vi "RT_NetworkStreams.vi"() -> ()   [LabVIEW 2025]
uses:
  <vilib>/dex/Flush And Wait Empty Condition.ctl
panel:
  out "error out 2":errorcluster
  out "error out":errorcluster
  out "Sinus RT":dbl[](graph)
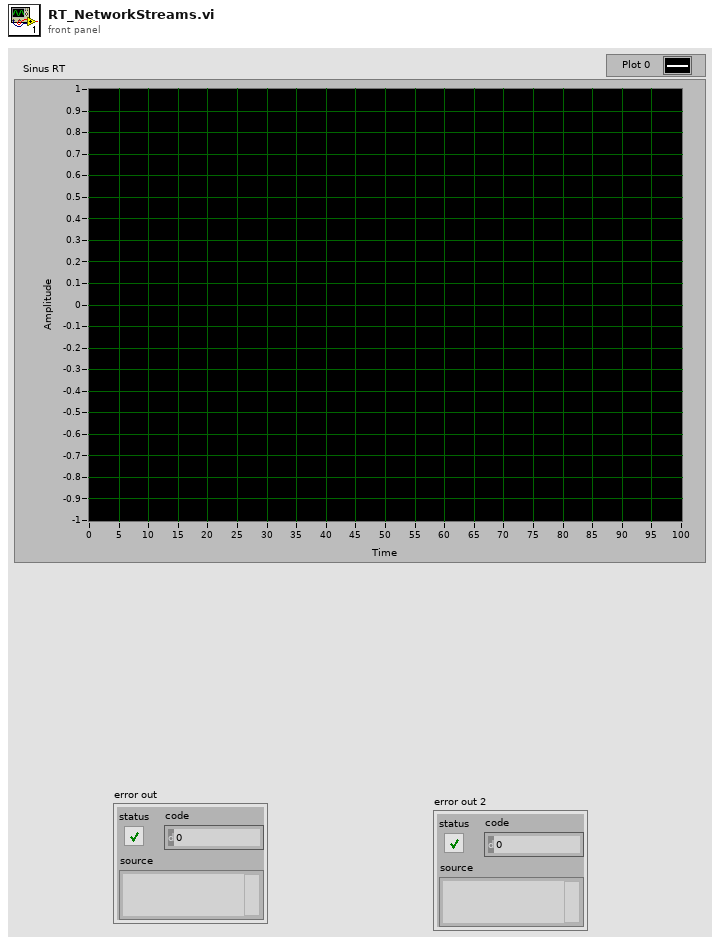
[diagram p1: front panel]
types:
  T1 = typedef "Flush And Wait Empty Condition.ctl" = u8
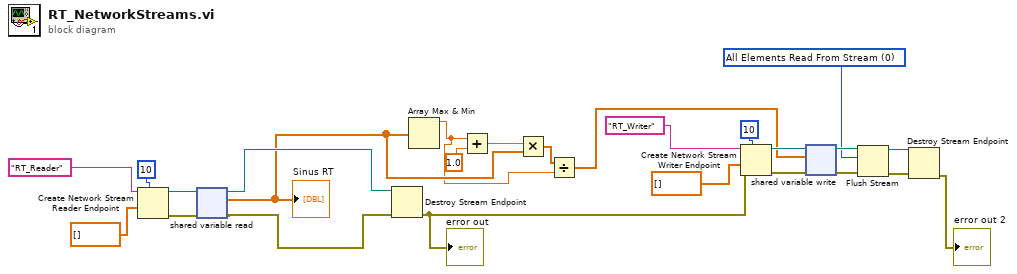
[diagram p0: block diagram]
diagram:
  w7 = T1 0 items=["All Elements Read From Stream", "All Elements Available for Reading"] ("wait condition")
  n1 = Create Network Stream Reader Endpoint(7:10 ("reader buffer size"), 9:dbl[] [], 11:"RT_Reader" ("reader name")) -> (0:w21:errorcluster, 3:w22:refnum<k21>)  [unwired: 4 in]
  n2 = shared-variable-read(w22, w21) -> (w20:refnum<k21>, w19:errorcluster, w4:dbl[])  [unwired: 1 in, 1 out]
  "Sinus RT" <- w4
  n3 = Destroy Stream Endpoint(8:w19, 11:w20) -> (0:w18:errorcluster)
  "error out" <- w18
  n4 = Array Max & Min(array=w4) -> (max value=w2:dbl)  [unwired: 3 out]
  n5 = Add(x=w2, y=1.0) -> (x+y=w5:dbl)
  n6 = Multiply(x=w5, y=w4) -> (x*y=w3:dbl[])
  n7 = Divide(x=w3, y=w2) -> (x/y=w1:dbl[])
  n8 = Create Network Stream Writer Endpoint(7:10 ("writer buffer size"), 8:w18, 9:dbl[] [], 11:"RT_Writer" ("writer name")) -> (0:w13:errorcluster, 3:w14:refnum<k21>)  [unwired: 3 in]
  n9 = shared-variable-write(w14, w13, w1) -> (w11:refnum<k21>, w12:errorcluster)  [unwired: 1 in, 1 out]
  n10 = Flush Stream(8:w12, 10:w7, 11:w11) -> (0:w9:errorcluster, 3:w10:refnum<k21>)  [unwired: 1 in, 1 out]
  n11 = Destroy Stream Endpoint(8:w9, 11:w10) -> (0:→"error out 2":errorcluster)
